vi "Get Path.vi"(6 "Strip lead \"/\" (F)":bool, 7 "Use base-path?":bool, 8 "error in (no error)":errorcluster, 11 "URI in":refnum<class "URI.lvclass">) -> (0 "error out":errorcluster, 2 "path":string, 3 "URI out":refnum<class "URI.lvclass">)   [LabVIEW 2013, in "openURI.lvlib" / "URI.lvclass"]
uses:
  URI.lvclass
  URI.lvclass/URI.ctl
  components/path/URI-Component.Path.lvclass
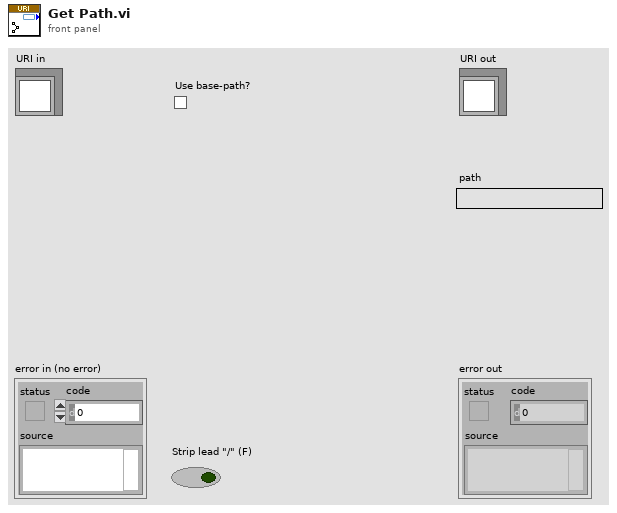
[diagram p1: front panel]
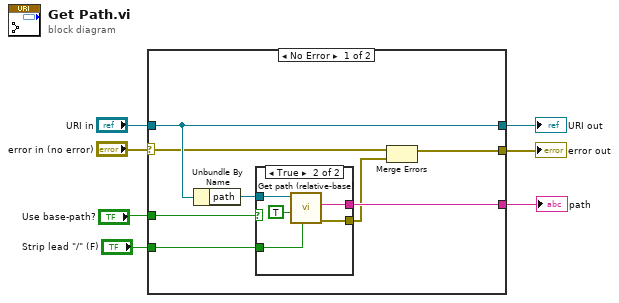
[diagram p0: block diagram]
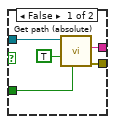
[diagram p2: hidden frame]
diagram:
  n1 = case shown="No Error" "error in (no error)" {
    selector: "error in (no error)" -> [w12 w27]
    tunnel: [w10 w27] -> w6
    tunnel: [w13 w26] -> w4
    tunnel: "URI in" -> [w13 w26]
    tunnel: [w14 _] -> w3
    tunnel: "Strip lead \"/\" (F)" -> [w9 _]
    tunnel: "Use base-path?" -> [w8 _]
    frame No Error {
      n2 = Unbundle By Name(w13) -> ("path"=w15:refnum<class "URI-Component.Path.lvclass">)
      n3 = case shown="True" w8 {
        tunnel: w15 -> [w20 w25]
        tunnel: [w19 w24] -> w14
        tunnel: [w18 w23] -> w11
        tunnel: w9 -> [w16 w22]
        frame False {
          n4 = call "Get path (absolute).vi"("Strip lead \"/\" (F)"=w16, "Encoded? (F)"=TRUE, "URI-Component.Path in"=w20) -> ("error out"=w18:errorcluster, "path-component"=w19:string)  [unwired: 6 in, 1 out]
        }
        frame True {
          n5 = call "Get path (relative-base).vi"("Strip lead \"/\" (F)"=w22, "Encoded? (F)"=TRUE, "URI-Component.Path in"=w25) -> ("error out"=w23:errorcluster, "relative-path"=w24:string)  [unwired: 5 in, 2 out]
        }
      }
      n6 = Merge Errors(w12, w11) -> (w10:errorcluster)
    }
    frame Error {
    }
  }
  "error out" <- w6
  "URI out" <- w4
  "path" <- w3
